vi "ASD Signal Triger Detection VI.vi"(8 "方向":enum16{"両方", "立ち上がり", "立ち下がり"}(ring), 9 "下閾値":dbl=1.0, 10 "上閾値":dbl=1.0, 11 "入力配列":dbl[](array[numeric])) -> (0 "開始":i32[](array[numeric]), 1 "立下り":i32[](array[numeric]), 2 "立ち上がり":i32[](array[numeric]), 3 "位置":i32[](array[numeric]))   [LabVIEW 2018]
panel:
  out "配列 2":bool[](array[boolean])
  out "配列":bool[](array[boolean])
  out ".not. x?":bool
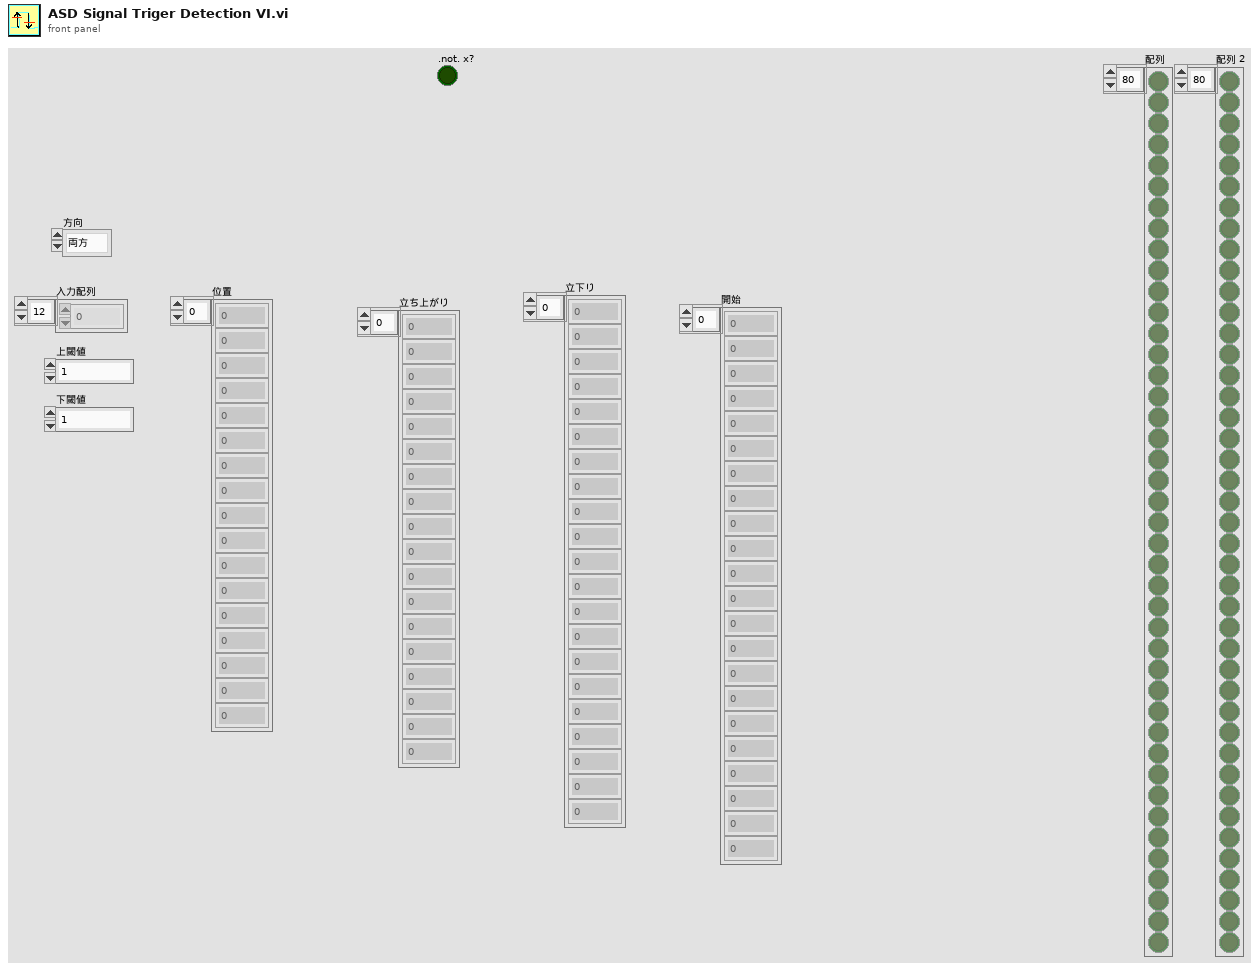
[diagram p1: front panel]
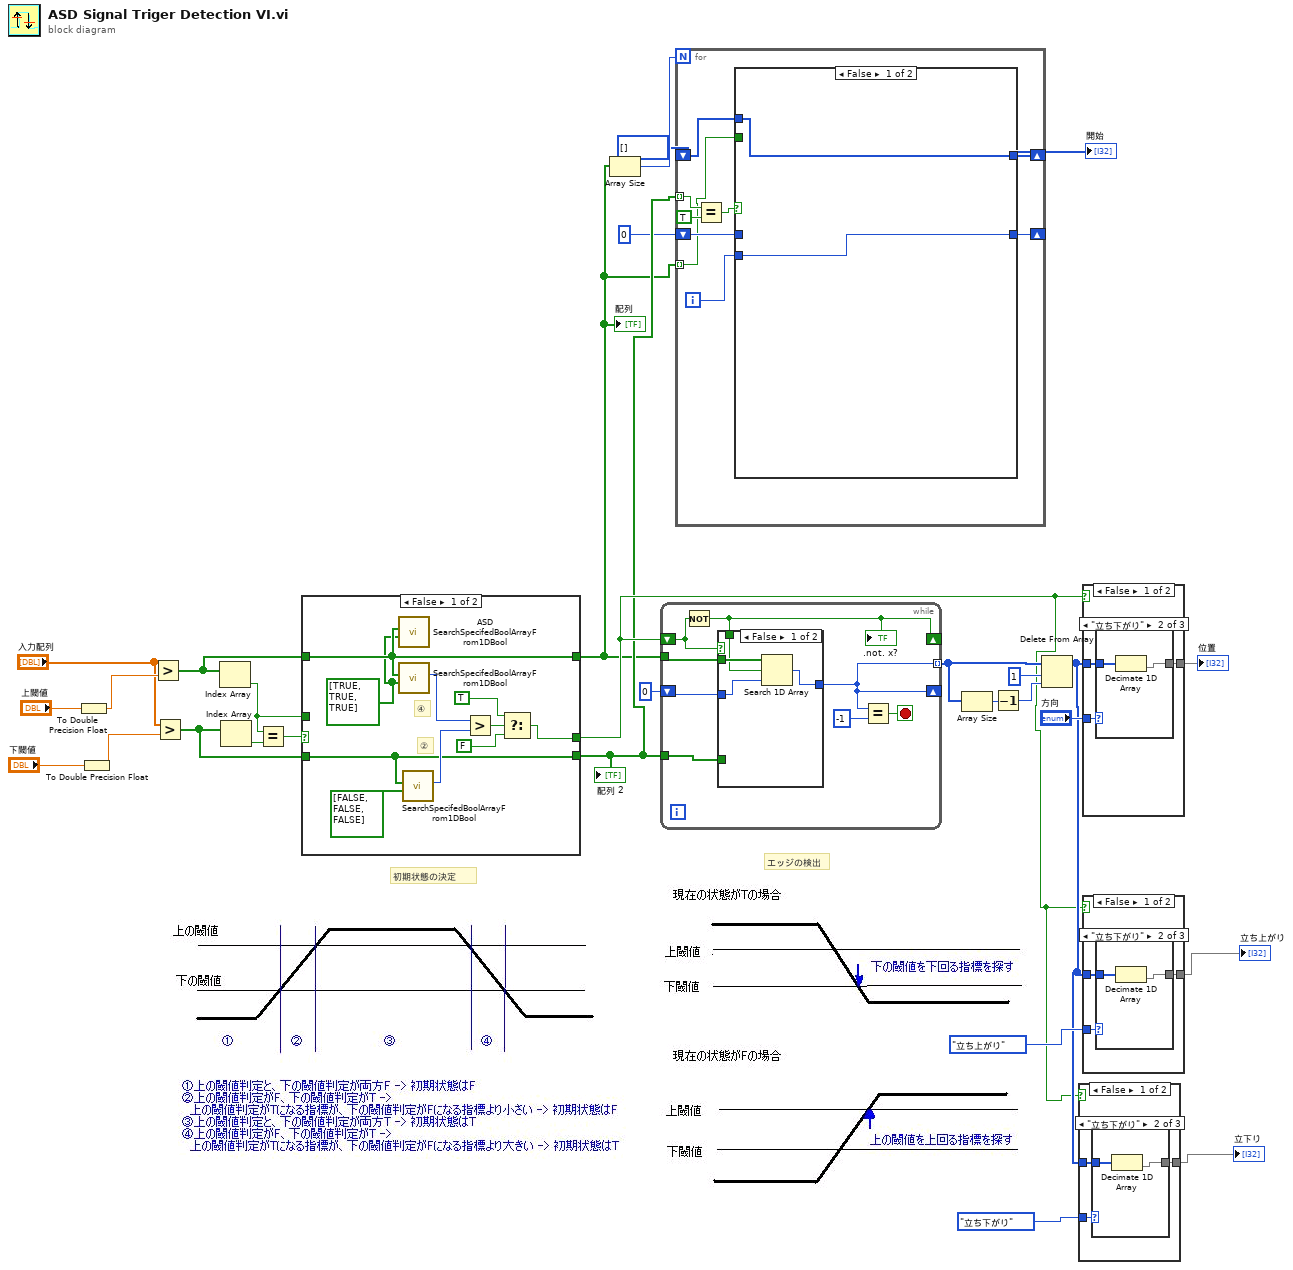
[diagram p0: block diagram]
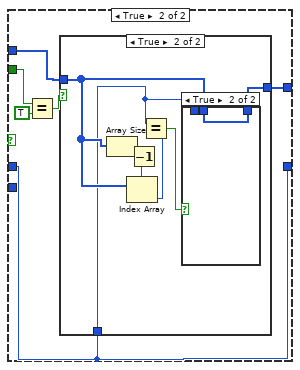
[diagram p2: hidden frame]
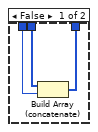
[diagram p4: hidden frame]
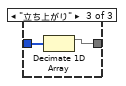
[diagram p6: hidden frame]
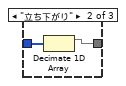
[diagram p8: hidden frame]
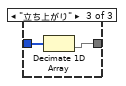
[diagram p9: hidden frame]
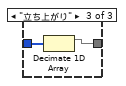
[diagram p11: hidden frame]
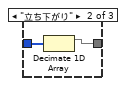
[diagram p13: hidden frame]
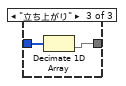
[diagram p14: hidden frame]
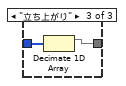
[diagram p17: hidden frame]
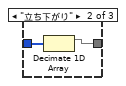
[diagram p19: hidden frame]
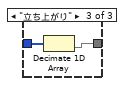
[diagram p20: hidden frame]
diagram:
  # "エッジの検出"
  # "初期状態の決定"
  n1 = To Double Precision Float(number="上閾値") -> (double precision float=w3:dbl)
  n2 = To Double Precision Float(number="下閾値") -> (double precision float=w2:dbl)
  n3 = Greater?(x="入力配列", y=w3) -> (0:w19:bool[])
  n4 = Greater?(x="入力配列", y=w2) -> (0:w18:bool[])
  n5 = Index Array(array=w19) -> (element=w16:bool)  [unwired: 1 in]
  n6 = Index Array(array=w18) -> (element=w21:bool)  [unwired: 1 in]
  n7 = Equal?(x=w16, y=w21) -> (x = y?=w20:bool)
  n8 = case shown="False" w20 {
    tunnel: [w36 w40] -> w10
    tunnel: w19 -> [w32 w42]
    tunnel: w18 -> [w33 w41]
    tunnel: [w32 w42] -> w7
    tunnel: [w33 w41] -> w8
    tunnel: w16 -> [_ w40]
    frame False {
      w31 = bool[] [TRUE, TRUE, TRUE] ("検索する配列")
      # "②"
      # "④"
      n9 = call "ASD SearchSpecifedBoolArrayFrom1DBool.vi"("検索する配列"=w31, "対象とする配列"=w32) -> ()  [unwired: 9 in, 1 out]
      n10 = call "SearchSpecifedBoolArrayFrom1DBool.vi"("検索する配列"=w31, "対象とする配列"=w32) -> ("指標"=w30:i32)  [unwired: 9 in]
      n11 = call "SearchSpecifedBoolArrayFrom1DBool.vi"("検索する配列"=bool[] [FALSE, FALSE, FALSE], "対象とする配列"=w33) -> ("指標"=w38:i32)  [unwired: 9 in]
      n12 = Greater?(x=w30, y=w38) -> (0:w37:bool)
      n13 = Select(t=TRUE ("ブール"), s=w37, f=FALSE ("ブール")) -> (s? t:f=w36:bool)
    }
    frame True {
      # "①と③"
    }
  }
  "配列" <- w7
  "配列 2" <- w8
  n14 = Array Size(array=w7) -> (size(s)=w9:i32)
  n15 = while {
    tunnel: w7 -> [w50]
    shift-right: [w43] -> _
    shift-left: w10 -> [w44]
    shift-right: [w48] -> _
    shift-left: 0 ("index of element") -> [w49]
    tunnel: [w48] -> w24 mode=indexing
    tunnel: w8 -> [w45]
    stop <- w46 stop-if-true
    n16 = Not(x=w44) -> (.not. x?=w43:bool)
    ".not. x?" <- w43
    n17 = case shown="False" w44 {
      tunnel: w50 -> [w54 _]
      tunnel: w49 -> [w52 w55]
      tunnel: [w51 w58] -> w48
      tunnel: w45 -> [_ w56]
      tunnel: w43 -> [w53 w57]
      frame False {
        n18 = Search 1D Array(1D array=w54, element=w53, start index (0)=w52) -> (index of element=w51:i32)
      }
      frame True {
        n19 = Search 1D Array(1D array=w56, element=w57, start index (0)=w55) -> (index of element=w58:i32)
      }
    }
    n20 = Equal?(x=w48, y=-1) -> (x = y?=w46:bool)
  }
  n21 = for {
    N: w9 -> [_]
    tunnel: w8 -> [w66] mode=indexing
    tunnel: w7 -> [w61] mode=indexing
    shift-right: [w63] -> _
    shift-left: 0 ("index of element") -> [w62]
    shift-right: [w60] -> w4
    shift-left: i32[] [] -> [w59]
    i -> [w64]
    n22 = Equal?(x=w66, y=TRUE) -> (x = y?=w67:bool)
    n23 = case shown="False" w67 {
      tunnel: w64 -> [w69 _]
      tunnel: [w69 w72] -> w63
      tunnel: w62 -> [_ w72]
      tunnel: w61 -> [_ w75]
      tunnel: [w68 w71] -> w60
      tunnel: w59 -> [w68 w70]
      frame False {
      }
      frame True {
        n24 = Equal?(x=w75, y=TRUE) -> (x = y?=w73:bool)
        n25 = case shown="True" w73 {
          tunnel: w72 -> [_ w77]
          tunnel: [w76 w78] -> w71
          tunnel: w70 -> [w76 w79]
          frame False {
          }
          frame True {
            n26 = Array Size(array=w79) -> (size(s)=w83:i32)
            n27 = Decrement(x=w83) -> (x-1=w81:i32)
            n28 = Index Array(array=w79, index=w81) -> (element=w82:i32)
            n29 = Equal?(x=w77, y=w82) -> (x = y?=w80:bool)
            n30 = case shown="True" w80 {
              tunnel: w79 -> [w86 w87]
              tunnel: [w85 w87] -> w78
              tunnel: w77 -> [w84 _]
              frame False {
                n31 = Build Array (concatenate)(w86, w84) -> (w85:i32[])
              }
              frame True {
              }
            }
          }
        }
      }
    }
  }
  "開始" <- w4
  n32 = Array Size(array=w24) -> (size(s)=w27:i32)
  n33 = Decrement(x=w27) -> (x-1=w28:i32)
  n34 = Delete From Array(array=w24, length=1 ("長さ"), index=w28) -> (array with subset deleted=w13:i32[])  [unwired: 1 out]
  n35 = case shown="False" w10 {
    tunnel: w13 -> [w88 w96]
    tunnel: enum16{"両方", "立ち上がり", "立ち下がり"}."立ち下がり" ("方向 3") -> [w90 w98]
    tunnel: [w89 w97] -> w12
    frame False {
      n36 = case shown="\"立ち下がり\"" w90 {
        tunnel: w88 -> [w91 w93 w95]
        tunnel: [w91 w92 w94] -> w89
        frame "両方", Default {
        }
        frame "立ち下がり" {
          n37 = Decimate 1D Array(w93) -> (w92:i32[])  [unwired: 1 out]
        }
        frame "立ち上がり" {
          n38 = Decimate 1D Array(w95) -> (w94:i32[])  [unwired: 1 out]
        }
      }
    }
    frame True {
      n39 = case shown="\"両方\", Default" w98 {
        tunnel: w96 -> [w99 w101 w103]
        tunnel: [w99 w100 w102] -> w97
        frame "両方", Default {
        }
        frame "立ち下がり" {
          n40 = Decimate 1D Array(w101) -> (w100:i32[])  [unwired: 1 out]
        }
        frame "立ち上がり" {
          n41 = Decimate 1D Array(w103) -> (w102:i32[])  [unwired: 1 out]
        }
      }
    }
  }
  "立下り" <- w12
  n42 = case shown="False" w10 {
    tunnel: w13 -> [w104 w112]
    tunnel: "方向" -> [w106 w114]
    tunnel: [w105 w113] -> w25
    frame False {
      n43 = case shown="\"立ち下がり\"" w106 {
        tunnel: w104 -> [w107 w109 w111]
        tunnel: [w107 w108 w110] -> w105
        frame "両方", Default {
        }
        frame "立ち下がり" {
          n44 = Decimate 1D Array(w109) -> (w108:i32[])  [unwired: 1 out]
        }
        frame "立ち上がり" {
          n45 = Decimate 1D Array(w111) -> (w110:i32[])  [unwired: 1 out]
        }
      }
    }
    frame True {
      n46 = case shown="\"両方\", Default" w114 {
        tunnel: w112 -> [w115 w117 w119]
        tunnel: [w115 w116 w118] -> w113
        frame "両方", Default {
        }
        frame "立ち下がり" {
          n47 = Decimate 1D Array(w117) -> (w116:i32[])  [unwired: 1 out]
        }
        frame "立ち上がり" {
          n48 = Decimate 1D Array(w119) -> (w118:i32[])  [unwired: 1 out]
        }
      }
    }
  }
  "位置" <- w25
  n49 = case shown="False" w10 {
    tunnel: w13 -> [w120 w128]
    tunnel: enum16{"両方", "立ち上がり", "立ち下がり"}."立ち上がり" ("方向 2") -> [w122 w130]
    tunnel: [w121 w129] -> w15
    frame False {
      n50 = case shown="\"立ち下がり\"" w122 {
        tunnel: w120 -> [w123 w125 w127]
        tunnel: [w123 w124 w126] -> w121
        frame "両方", Default {
        }
        frame "立ち下がり" {
          n51 = Decimate 1D Array(w125) -> (w124:i32[])  [unwired: 1 out]
        }
        frame "立ち上がり" {
          n52 = Decimate 1D Array(w127) -> (w126:i32[])  [unwired: 1 out]
        }
      }
    }
    frame True {
      n53 = case shown="\"両方\", Default" w130 {
        tunnel: w128 -> [w131 w133 w135]
        tunnel: [w131 w132 w134] -> w129
        frame "両方", Default {
        }
        frame "立ち下がり" {
          n54 = Decimate 1D Array(w133) -> (w132:i32[])  [unwired: 1 out]
        }
        frame "立ち上がり" {
          n55 = Decimate 1D Array(w135) -> (w134:i32[])  [unwired: 1 out]
        }
      }
    }
  }
  "立ち上がり" <- w15
